vi "GOOP_LVClass_Item_Init.vi"(11 "Object":u64) -> ()   [LabVIEW 2020]
doc: "Copyright (c) 2010 Symbio (www.symbio.com). All rights reserved."
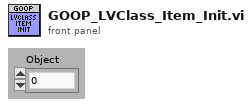
[diagram p1: front panel]
types:
  T1 = typedef "ItemRef.ctl" = u64
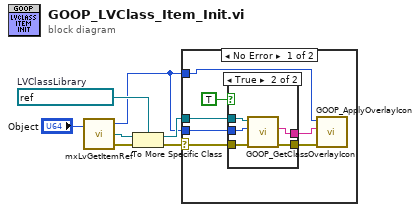
[diagram p0: block diagram]
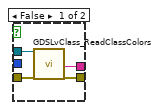
[diagram p2: hidden frame]
diagram:
  w4 = refnum<vi> refnum  # LVClassLibrary
  n1 = call <resource>:"mxLvGetItemRef.vi"("Item"="Object") -> ("Item"=w1:T1, "Item Refnum"=w6:refnum<vi>, "error out"=w3:errorcluster)  [unwired: 1 in]
  n2 = To More Specific Class(target class=w4, reference=w6, error in=w3) -> (specific class reference=w5:refnum<vi>, error out=w2:errorcluster)
  n3 = case shown="No Error" w2 {
    selector: w2 -> [w10 _]
    tunnel: w1 -> [w14 _]
    tunnel: w5 -> [w11 _]
    tunnel: w1 -> [w9 _]
    frame No Error {
      n4 = case shown="True" TRUE {
        tunnel: [w15 w23] -> w13
        tunnel: [w16 w19] -> w12
        tunnel: w11 -> [w17 w22]
        tunnel: w10 -> [w18 w21]
        tunnel: w9 -> [_ w20]
        frame False {
          n5 = call "GDSLvClass_ReadClassColors.vi"("Library Refnum"=w17, "error in (no error)"=w18) -> ("ClassItemIconName(NoExtension)"=w16:string, "error out"=w15:errorcluster)  [unwired: 12 in, 4 out]
        }
        frame True {
          n6 = call "GOOP_GetClassOverlayIcon.vi"("error in (no error)"=w21, "Item"=w20, "LVClassLibrary in"=w22) -> ("error out"=w23:errorcluster, "IconName"=w19:string)  [unwired: 6 in, 1 out]
        }
      }
      n7 = call "GOOP_ApplyOverlayIcon.vi"("error in (no error)"=w13, "IconName(NoPngExtension)"=w12, "Object"=w14) -> ()  [unwired: 8 in, 1 out]
    }
    frame Error {
    }
  }
